vi "Read MCP Request Metadata.vi"(8 "error in":errorcluster, 11 "request":string) -> (0 "error out":errorcluster, 3 "MCP Request Metadata":T1)   [LabVIEW 2020, in "MCP Server.lvlib"]
doc: "Reads what Handle MCP Request.vi needs to know about one request body and returns it as MCP Request Metadata.ctl: the method, the id as JSON text (null when missing), the io.modelcontextprotocol/protocolVersion and clientCapabilities of params._meta, params.uri for resources/read and params.name otherwise, the elicitation capability, and params.inputResponses ({} when missing).\n\nIt also decides the era, per request and without session state: a JSON object whose params._meta carries io.modelcontextprotocol/protocolVersion is MODERN (MCP 2026-07-28), unless its method is initialize. Everything else is LEGACY. A modern server/discover request with an id is marked discover, a JSON array is marked batch.\n\nA missing item is not an error of the request: the JSONtext errors are merged and cleared here. error in is passed through unchanged and does not stop the reading."
uses:
  MCP Server.lvlib
  MCP Request Metadata.ctl
  dbf4d01f-6e64-41ba-a74b-6a94db3b7925.vi
  bd13702f-2d9e-4981-9e4d-410909a23b11.vi
  3d72e98d-08b2-47da-83fb-3b5a902f0d10.vi
  50f52288-58a0-4d80-a697-5b8cd9dea1bd.vi
  <vilib>/JDP Science/JSONtext/Next JSON Value.vi
  <vilib>/JDP Science/JSONtext/String Subset.vi
  <vilib>/JDP Science/JSONtext/Parsing/Advance past next JSON Value (inlined COPY).vi
  <vilib>/JDP Science/JSONtext/Parsing/Advance past whitespace.vi
  <vilib>/JDP Science/JSONtext/Parsing/Advance past String.vi
  <vilib>/JDP Science/JSONtext/Parsing/Advance past Number.vi
  <vilib>/JDP Science/JSONtext/Parsing/Advance past Line Ending.vi
  <vilib>/JDP Science/JSONtext/Parsing/Parse Full Path or Item Name.vi
  <vilib>/JDP Science/JSONtext/Parsing/Advance past Array.vi
  <vilib>/JDP Science/JSONtext/Parsing/Advance past Object.vi
  <vilib>/JDP Science/JSONtext/support/Error Cluster From Code.vi
  <vilib>/JDP Science/JSONtext/Offset/Find Item Locations by Path.vi
  <vilib>/JDP Science/JSONtext/JSON text to Variant.vi
  <vilib>/JDP Science/JSONtext/LVClass Serializer/JSONtext LVClass Serializer.lvclass
  <vilib>/JDP Science/JSONtext/JSONtext.lvlib
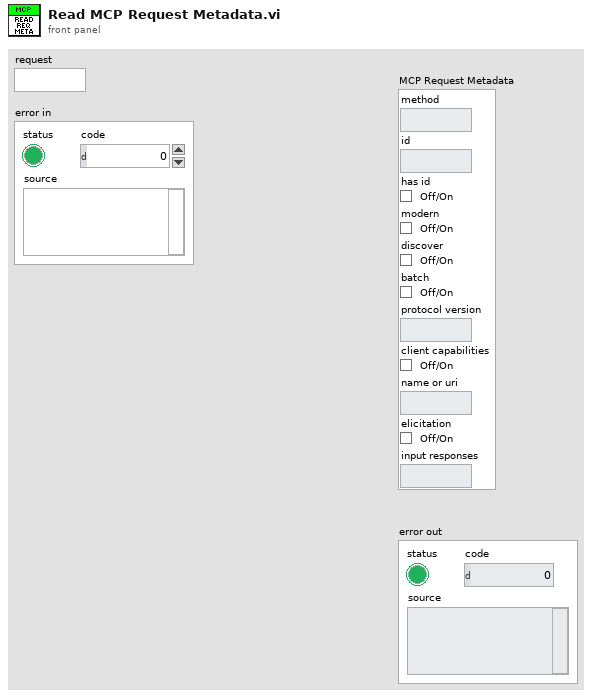
[diagram p1: front panel]
types:
  T1 = typedef "MCP Server.lvlib/MCP Request Metadata.ctl" = cluster{"method":string, "id":string, "has id":bool, "modern":bool, "discover":bool, "batch":bool, "protocol version":string, "client capabilities":bool, "name or uri":string, "elicitation":bool, "input responses":string}
  T2 = typedef "JSONtext.lvlib/JSON Value Type.ctl" = enum16{"Not a JSON Value", "JSON Object", "JSON Array", "String", "Number", "true", "false", "null"}
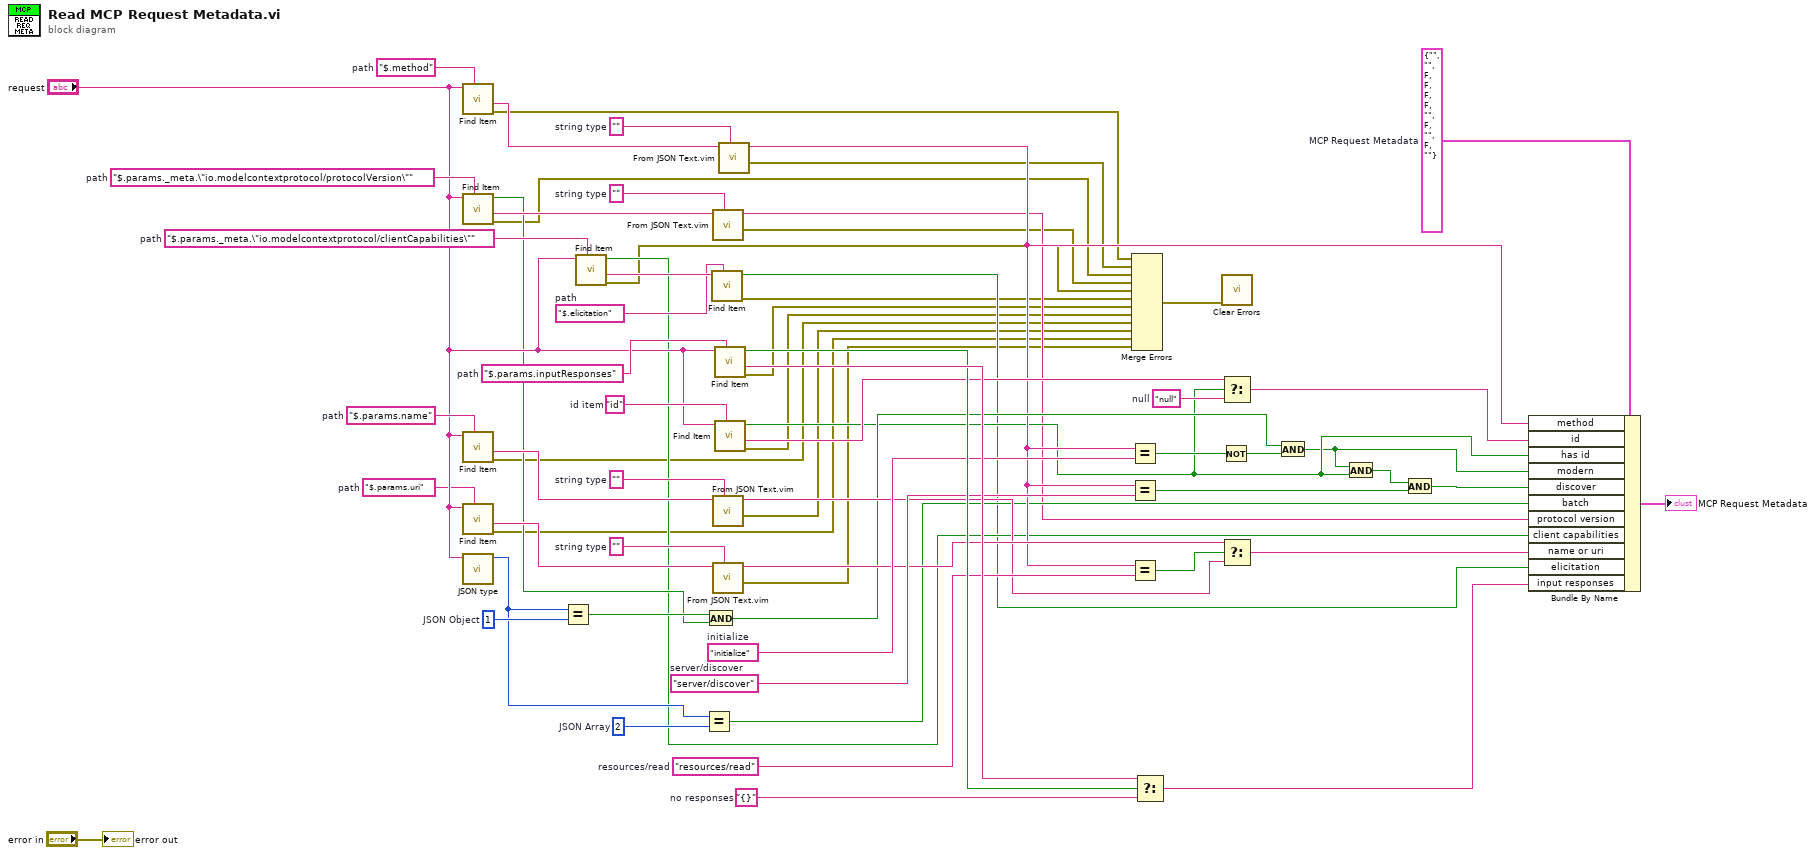
[diagram p0: block diagram]
diagram:
  w16 = T1 {"method"="", "id"="", "has id"=FALSE, "modern"=FALSE, "discover"=FALSE, "batch"=FALSE, "protocol version"="", "client capabilities"=FALSE, "name or uri"="", "elicitation"=FALSE, "input responses"=""}  # MCP Request Metadata
  w36 = "server/discover"  # server/discover
  w41 = ""  # string type
  w59 = "$.params.uri"  # path
  w43 = ""  # string type
  w61 = "$.params.name"  # path
  w37 = "resources/read"  # resources/read
  w38 = "initialize"  # initialize
  w45 = "null"  # null
  w62 = "id"  # id item
  w47 = "{}"  # no responses
  w63 = "$.params.inputResponses"  # path
  w50 = "$.elicitation"  # path
  w64 = "$.params._meta.\"io.modelcontextprotocol/clientCapabilities\""  # path
  w52 = ""  # string type
  w65 = "$.params._meta.\"io.modelcontextprotocol/protocolVersion\""  # path
  w54 = ""  # string type
  w66 = "$.method"  # path
  w56 = u16 2  # JSON Array
  w58 = u16 1  # JSON Object
  n1 = call <vilib>:"Find Item.vi"("$Path or Item Name"=w66, "JSON"="request") -> ("error out"=w15:errorcluster, "<JSON>"=w55:string)  [unwired: 6 in, 2 out]
  n2 = call <vilib>:"Find Item.vi"("$Path or Item Name"=w65, "JSON"="request") -> ("error out"=w13:errorcluster, "<JSON>"=w53:string, "Found"=w39:bool)  [unwired: 6 in, 1 out]
  n3 = call <vilib>:"Find Item.vi"("$Path or Item Name"=w61, "JSON"="request") -> ("error out"=w7:errorcluster, "<JSON>"=w44:string)  [unwired: 6 in, 2 out]
  n4 = call <vilib>:"Find Item.vi"("$Path or Item Name"=w59, "JSON"="request") -> ("error out"=w5:errorcluster, "<JSON>"=w42:string)  [unwired: 6 in, 2 out]
  n5 = call <vilib>:"JSON type.vi"("JSON"="request") -> ("JSON Value Type"=w57:T2)  [unwired: 9 in, 1 out]
  n6 = Equal?(x=w57, y=w58) -> (x = y?=w40:bool)
  n7 = call <vilib>:"Find Item.vi"("$Path or Item Name"=w64, "JSON"="request") -> ("error out"=w11:errorcluster, "<JSON>"=w51:string, "Found"=w20:bool)  [unwired: 6 in, 1 out]
  n8 = Equal?(x=w57, y=w56) -> (x = y?=w22:bool)
  n9 = And(x=w40, y=w39) -> (x .and. y?=w31:bool)
  n10 = call <vilib>:"Find Item.vi"("$Path or Item Name"=w50, "JSON"=w51) -> ("error out"=w10:errorcluster, "Found"=w18:bool)  [unwired: 6 in, 2 out]
  n11 = call "From JSON Text.vim"("Data Type and Default Value"=w52, "JSON"=w53) -> ("error out"=w12:errorcluster, "Data out"=w21:string)  [unwired: 8 in]
  n12 = call "From JSON Text.vim"("Data Type and Default Value"=w43, "JSON"=w44) -> ("error out"=w6:errorcluster, "Data out"=w32:string)  [unwired: 8 in]
  n13 = call "From JSON Text.vim"("Data Type and Default Value"=w41, "JSON"=w42) -> ("error out"=w4:errorcluster, "Data out"=w34:string)  [unwired: 8 in]
  n14 = call <vilib>:"Find Item.vi"("$Path or Item Name"=w63, "JSON"="request") -> ("error out"=w9:errorcluster, "<JSON>"=w49:string, "Found"=w48:bool)  [unwired: 6 in, 1 out]
  n15 = call <vilib>:"Find Item.vi"("$Path or Item Name"=w62, "JSON"="request") -> ("error out"=w8:errorcluster, "<JSON>"=w46:string, "Found"=w25:bool)  [unwired: 6 in, 1 out]
  n16 = call "From JSON Text.vim"("Data Type and Default Value"=w54, "JSON"=w55) -> ("error out"=w14:errorcluster, "Data out"=w27:string)  [unwired: 8 in]
  n17 = Equal?(x=w27, y=w38) -> (x = y?=w35:bool)
  n18 = Equal?(x=w27, y=w36) -> (x = y?=w28:bool)
  n19 = Equal?(x=w27, y=w37) -> (x = y?=w33:bool)
  n20 = Merge Errors(w15, w14, w13, w12, w11, w10, w9, w8, w7, w6, w5, w4) -> (w3:errorcluster)
  n21 = Select(t=w49, s=w48, f=w47) -> (s? t:f=w17:string)
  n22 = Not(x=w35) -> (.not. x?=w30:bool)
  n23 = call <vilib>:"Clear Errors.vi"("error in (no error)"=w3) -> ()  [unwired: 5 in, 2 out]
  n24 = Select(t=w46, s=w25, f=w45) -> (s? t:f=w26:string)
  n25 = Select(t=w34, s=w33, f=w32) -> (s? t:f=w19:string)
  n26 = And(x=w31, y=w30) -> (x .and. y?=w24:bool)
  n27 = And(x=w24, y=w25) -> (x .and. y?=w29:bool)
  n28 = And(x=w29, y=w28) -> (x .and. y?=w23:bool)
  n29 = Bundle By Name(cluster=w16, "method"=w27, "id"=w26, "has id"=w25, "modern"=w24, "discover"=w23, "batch"=w22, "protocol version"=w21, "client capabilities"=w20, "name or uri"=w19, "elicitation"=w18, "input responses"=w17) -> (→"MCP Request Metadata":T1)
  "error out" <- "error in"
